vi "{TMPL} MAIN - App.vi"() -> ()   [LabVIEW 2023, in "TLB` InstStu GPlugin Template.lvlib" / "{TMPL} TLB`.lvclass"]
uses:
  {TMPL} TLB`.lvclass
  Application Components/Trigger API/System Trigger.ctl
  State Machine/State.ctl
  Core Components/Error Handler/TLB` Error Handler.lvclass
  Application Components/Configuration/{TMPL} Station Configuration.lvclass
  {TMPL} TLB`.lvclass/{TMPL} TLB`.ctl
  Application Components/InstStuGPluginSDK/Plugin Events.ctl
  Application Components/InstStuGPluginSDK/Plugin Events Enum.ctl
  <vilib>/Utility/error.llb/Error Cluster From Error Code.vi
  <vilib>/ErrorRing/Error Ring.xnode
  Application Components/Trigger API/{TMPL} Trigger API.lvlib
  TLB` InstStu GPlugin Template.lvlib
  Core Components/Actions/Actions.lvlib
  Core Components/Dependencies/TLB`_Dependencies.lvlib
  Application Components/UI/ScrollZoomGraphChart/ScrollZoomGraphChart.lvclass
  Application Components/InstStuGPluginSDK/Plugin Session.lvclass
  Application Components/InstStuGPluginSDK/InstrumentStudio Plugin SDK.lvlib
  <vilib>/Utility/LVLibp/NI_PackedLibraryUtility.lvlib
panel:
  in  "Session Id":u64
  out "top banner":u32(colorbox)=44412
  out "iq graph":waveform(sgl)[](graph) caption="Q Data"
  out "iq graph 2":waveform(sgl)[](graph) caption="Q Data"
  out "iq graph 3":waveform(sgl)[](graph) caption="Q Data"
  out "iq graph 4":waveform(sgl)[](graph) caption="Q Data"
  in  "RESOURCE NAME":refnum<visa-resource-name>
  in  "error":bool
  out "error background":u32(colorbox)=15461355
  in  "settings gear":bool
  in  "connect":bool
  in  "run":bool
  in  "single":bool
  out "title":string="INST STU GPLUGIN`"
  out "error out":errorcluster
  in  "digital offset":dbl caption="DIGITAL OFFSET" format="%1_3p"
  in  "digital gain":dbl=-10.0 caption="DIGITAL GAIN" format="%1_3p dB"
  in  "finite records?":bool=TRUE
  in  "iq rate":dbl=2160000000.0 caption="IQ  RATE" format="%1_6p samples/sec"
  in  "no of samples":u64=1000 caption="NO. SAMPLES"
  in  "no of records":u64=25 caption="NO. RECORDS"
  in  "finite samples?":bool=TRUE
  in  "acq sample rate":dbl=2160000000.0 caption="ACQ SAMPLE RATE" format="%1_6p samples/sec"
  out "State":string="<Shutdown> "
  out "Status":string
  # "Section  A"
  # "Section B"
  # "Category A"
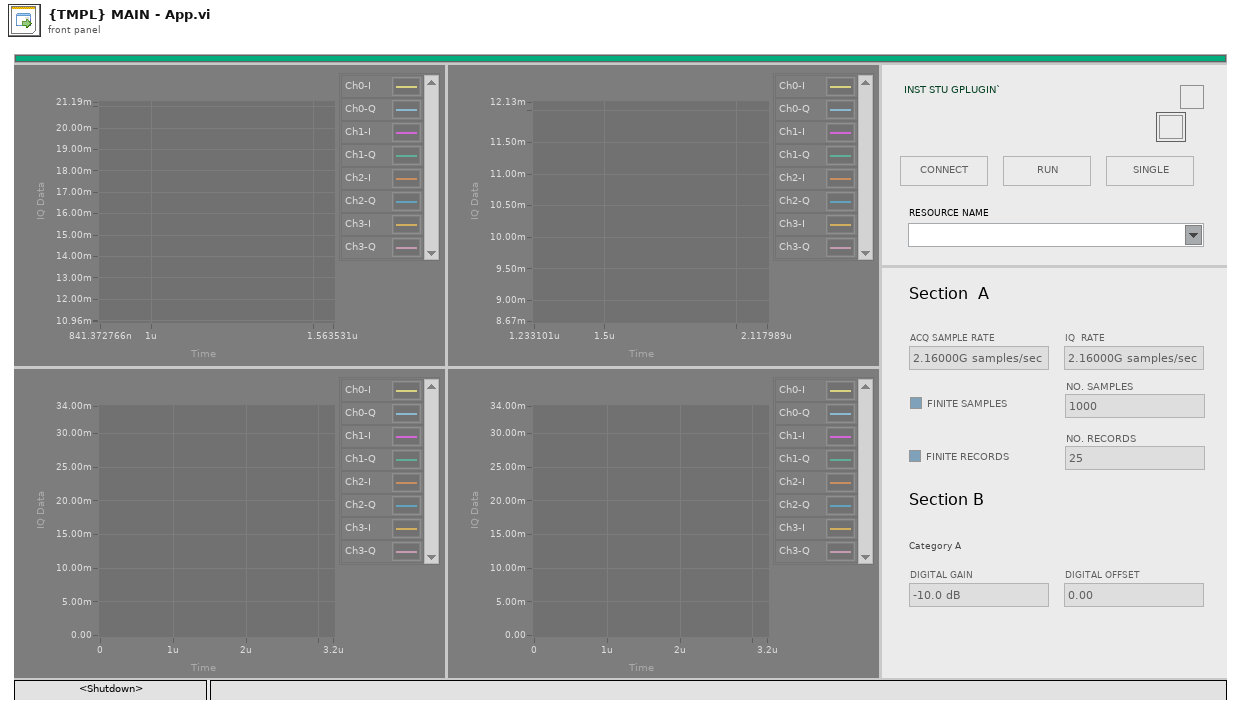
[diagram p1: front panel]
types:
  T1 = typedef "TLB` InstStu GPlugin Template.lvlib/{TMPL} TLB`.lvclass/State.ctl" = enum16{"<Startup>", "Idle", "Connected", "Monitoring", "<Shutdown>", "<Error>"}
  T2 = enum16{"Close Display", "Clear References", "Close Error Handler"}
  T3 = enum16{"Clear SR", "Set Display", "Set Shifter", "Initialize Events", "Init Q"}
  T4 = typedef "TLB` InstStu GPlugin Template.lvlib/{TMPL} Trigger API.lvlib/System Trigger.ctl" = enum16{"<None>", "Connect", "Start Acquisition", "Stop Acquisition", "Disconnect", "Load Configuration", "Save Configuration", "<Return to Safe State Actions>", "<Cache User Parameters>", "<Close Application>", "<Error>"}
  T5 = refnum<class "{TMPL} Station Configuration.lvclass">
  T6 = typedef "TLB` InstStu GPlugin Template.lvlib/InstrumentStudio Plugin SDK.lvlib/Plugin Events.ctl" = cluster{"Shutdown":refnum<user-event>, "Project Saved":refnum<user-event>, "Stop All Outputs":refnum<user-event>, "Generic Message":refnum<user-event>}
  T7 = typedef "TLB` InstStu GPlugin Template.lvlib/_UI CORE Event References.ctl" = cluster{"Exit Event":refnum<user-event>, "State Indicator":refnum<user-event>, "Status Indicator":refnum<user-event>}
  T8 = typedef "TLB` InstStu GPlugin Template.lvlib/_UI APP Event References.ctl" = cluster{"Exit Event":refnum<user-event>}
  T9 = typedef "TLB` InstStu GPlugin Template.lvlib/InstrumentStudio Plugin SDK.lvlib/Plugin Events Enum.ctl" = enum16{"Shutdown", "Project Saved", "Stop All Outputs", "Generic Message"}
  T10 = typedef "TLB` InstStu GPlugin Template.lvlib/InstrumentStudio Plugin SDK.lvlib/Panel Size.ctl" = enum32{"Large", "Small"}
  T11 = enum32{"Invalid", "Standard", "Closed", "Hidden", "Minimized", "Maximized"}
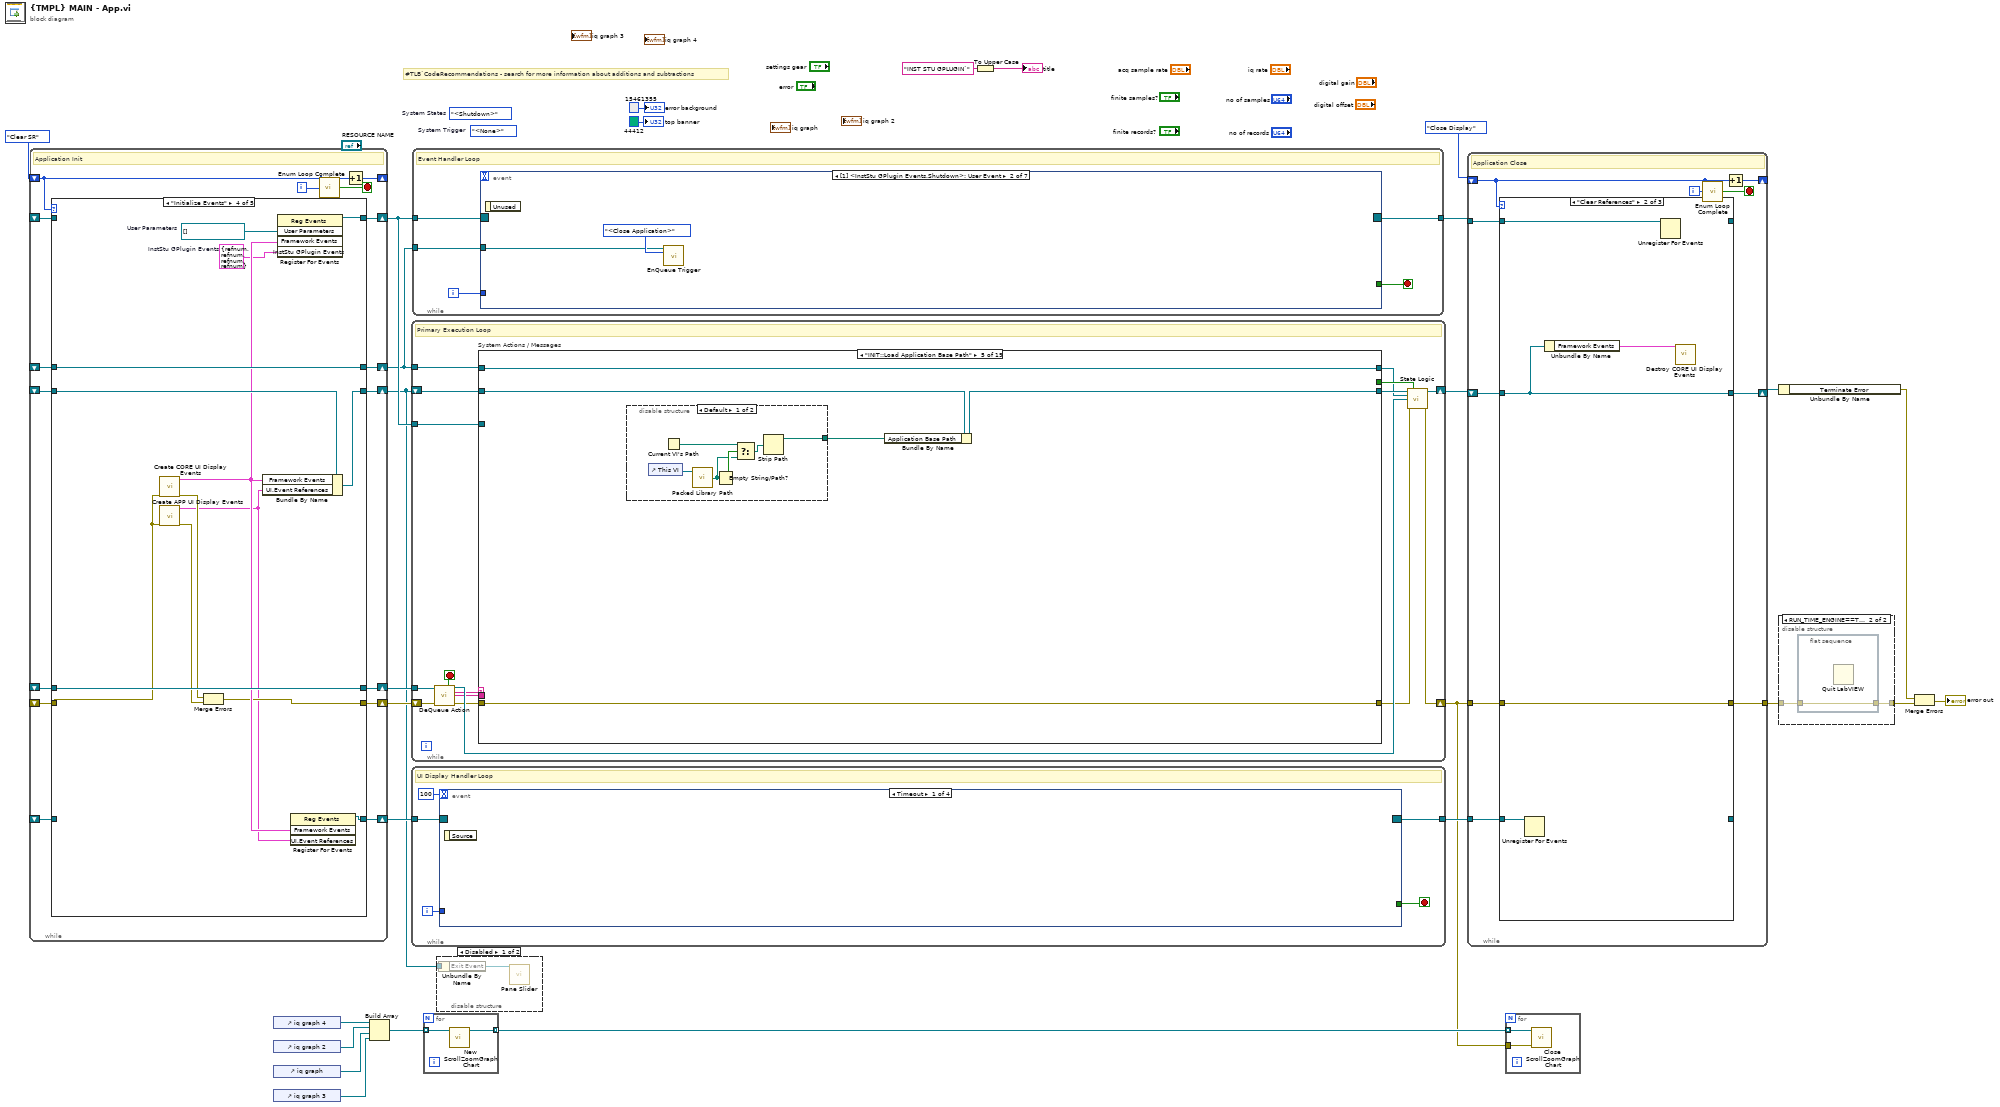
[diagram p0: block diagram]
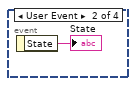
[diagram p3: hidden frame]
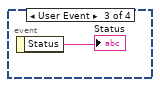
[diagram p4: hidden frame]
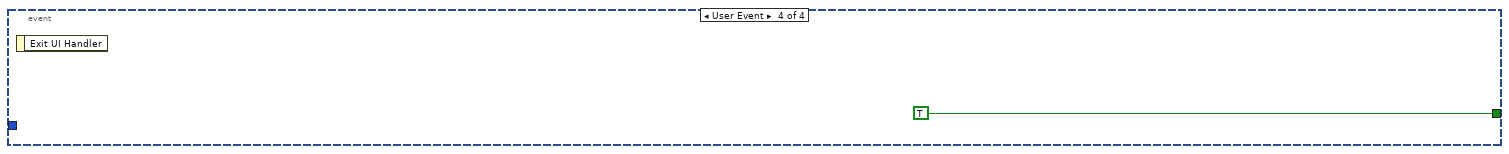
[diagram p5: hidden frame]
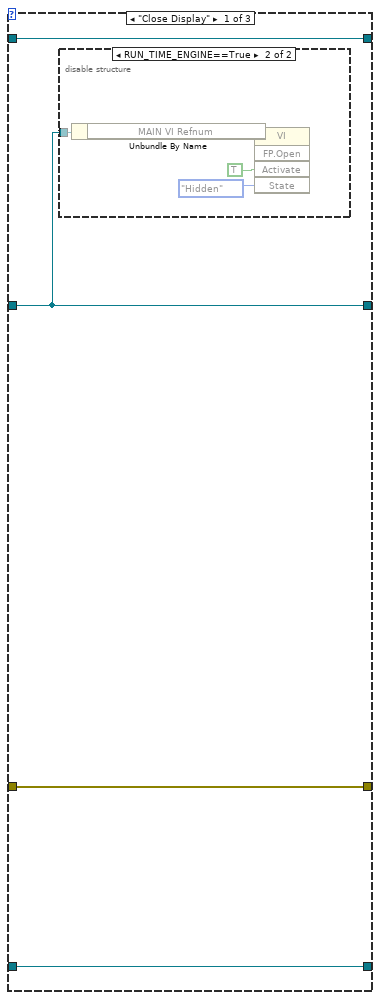
[diagram p7: hidden frame]
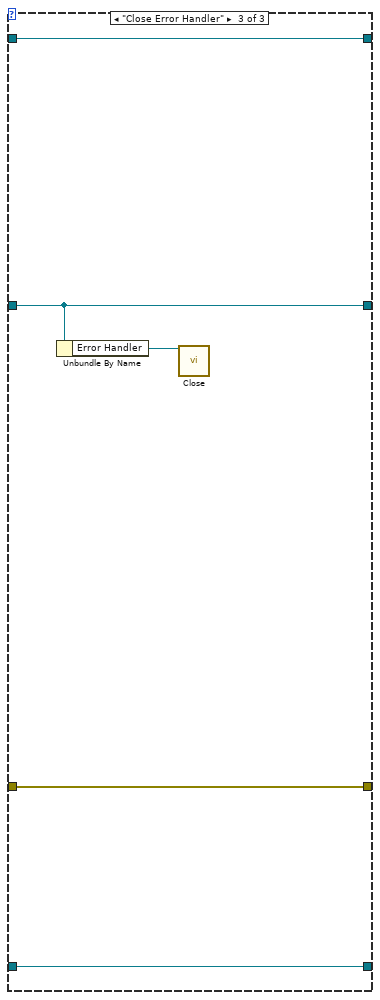
[diagram p9: hidden frame]
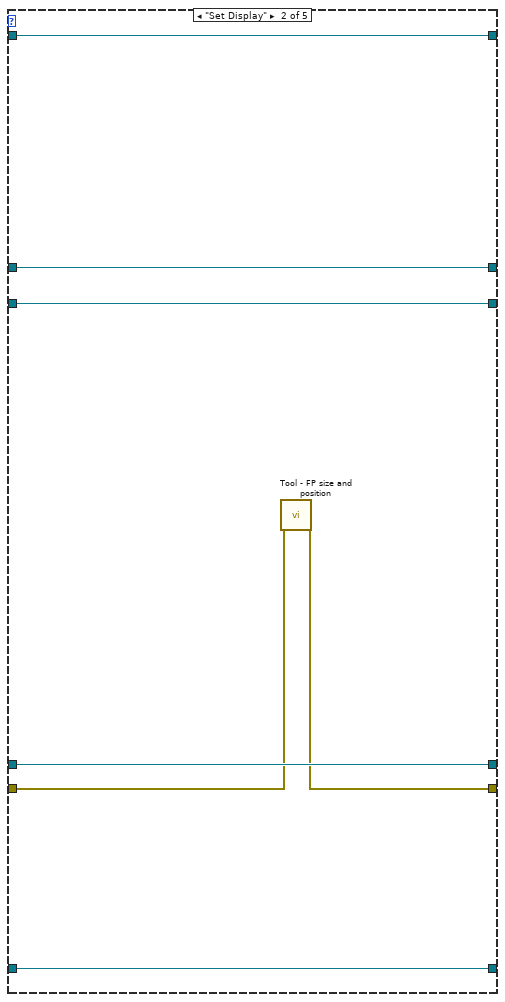
[diagram p11: hidden frame]
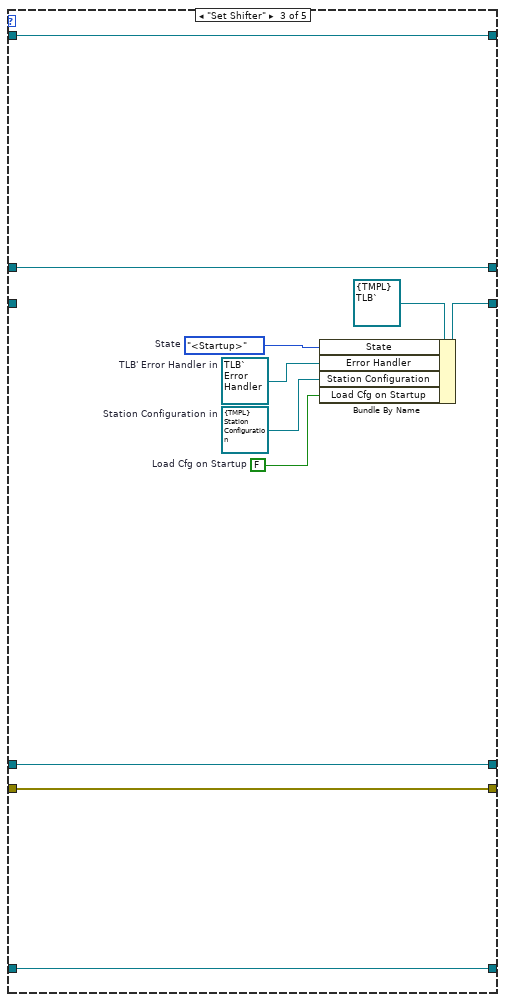
[diagram p12: hidden frame]
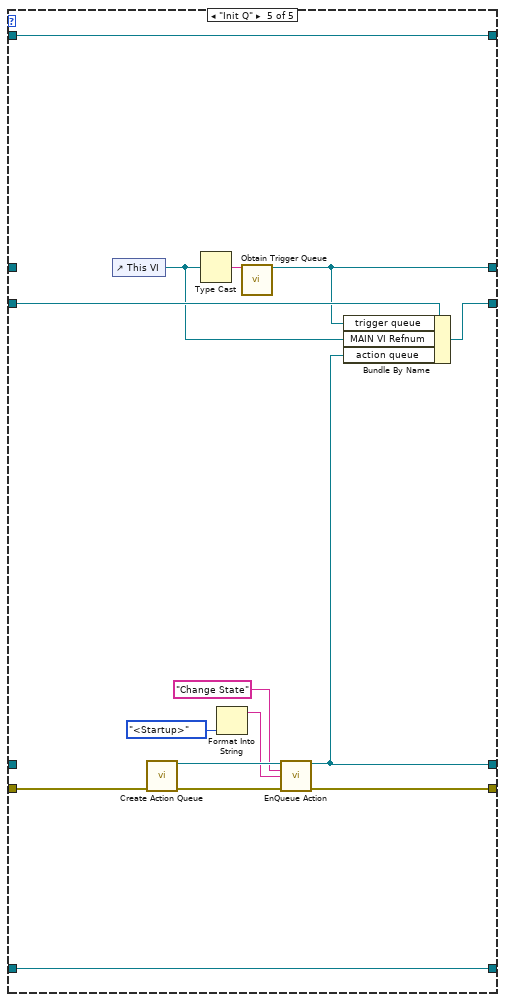
[diagram p13: hidden frame]
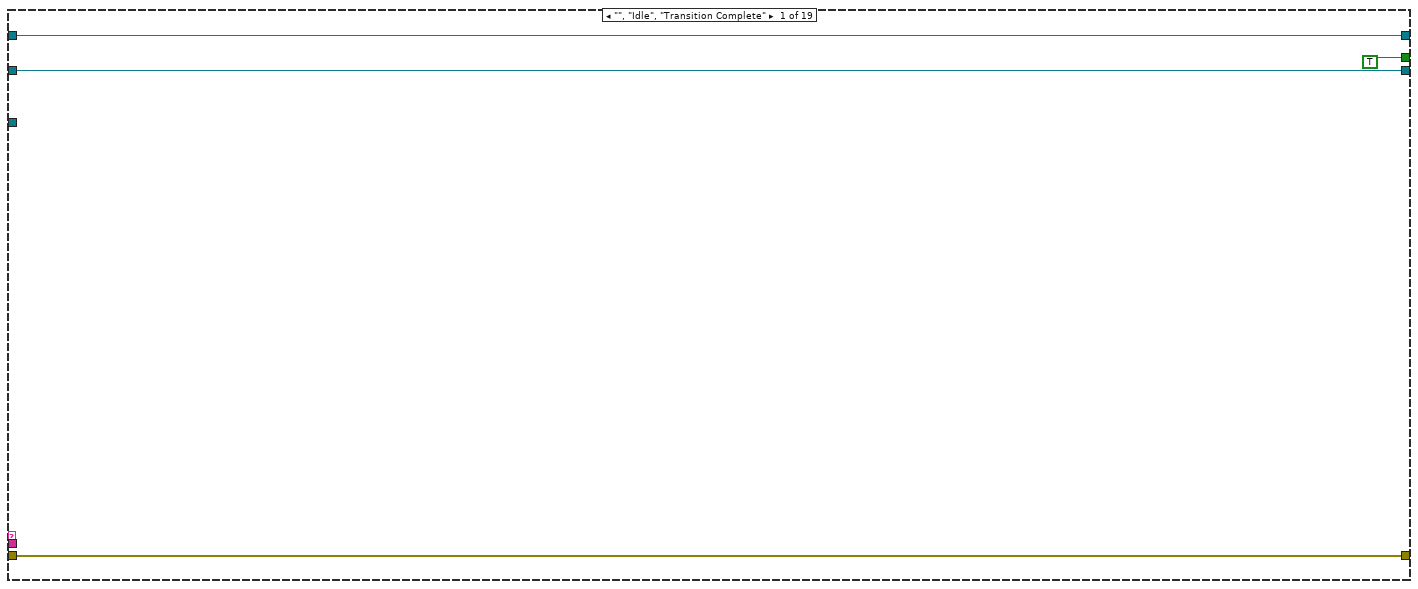
[diagram p14: hidden frame]
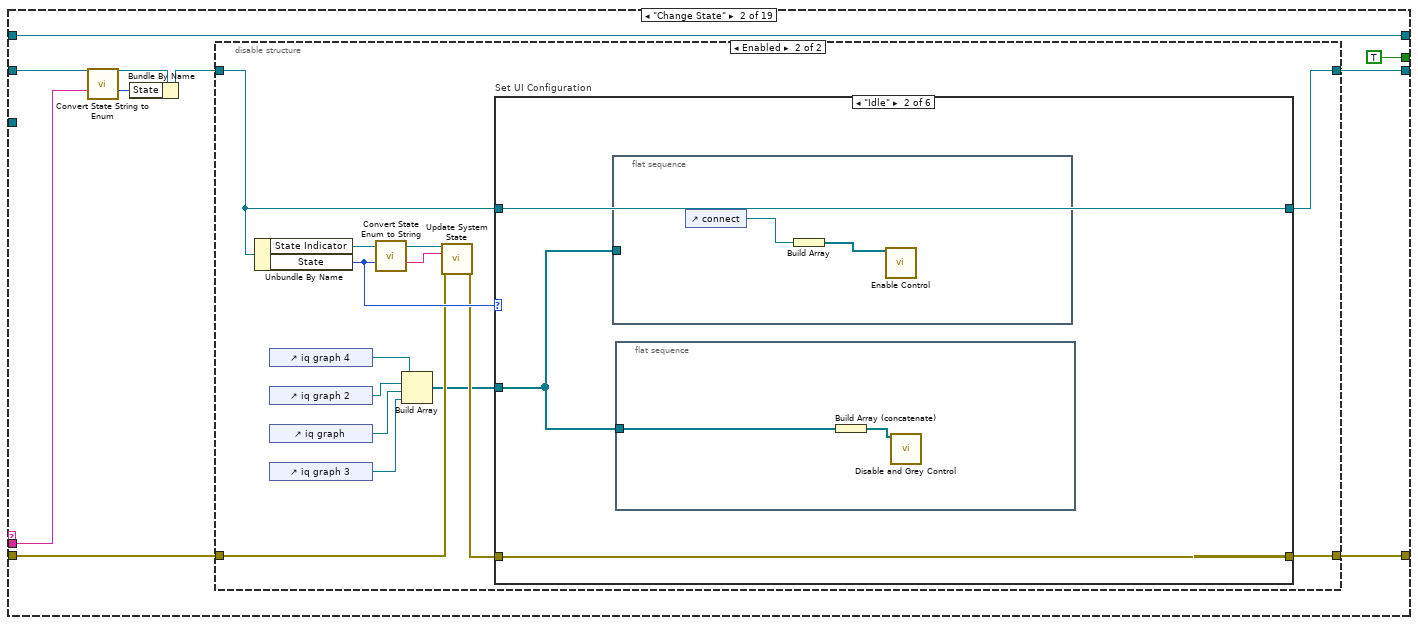
[diagram p15: hidden frame]
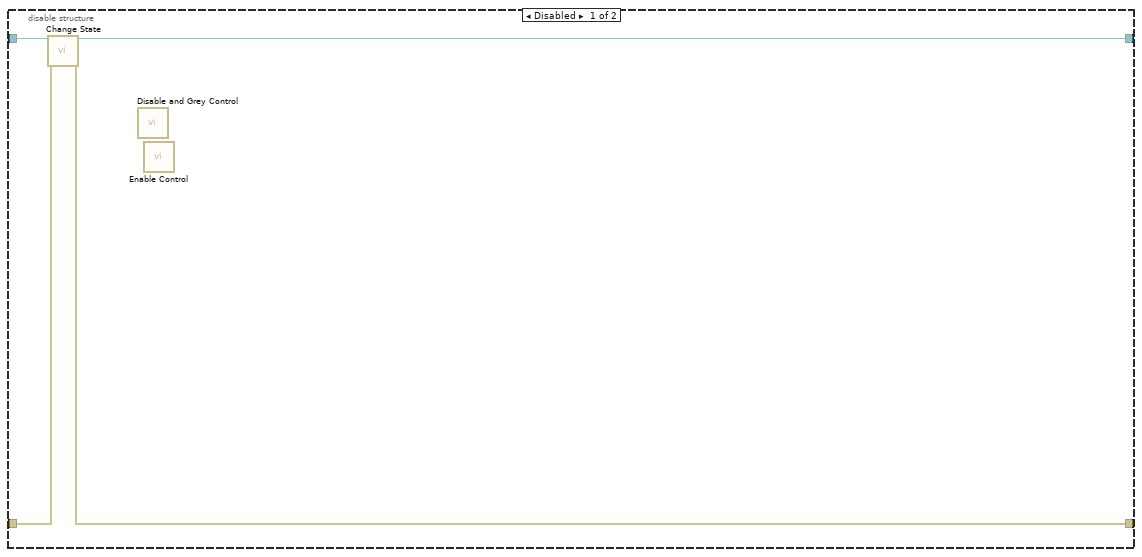
[diagram p16: hidden frame]
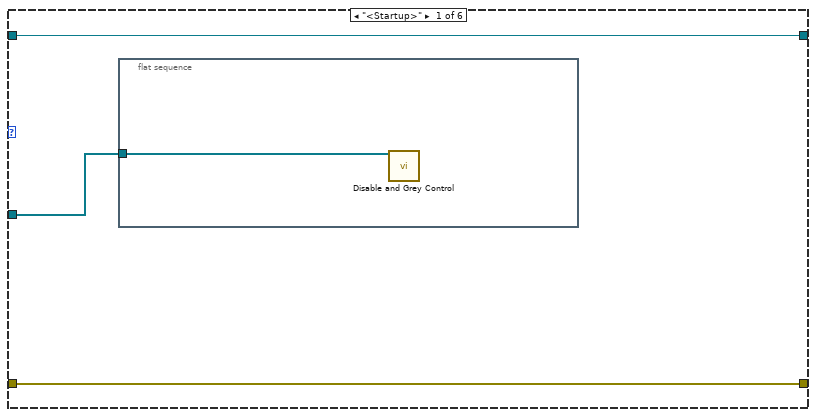
[diagram p17: hidden frame]
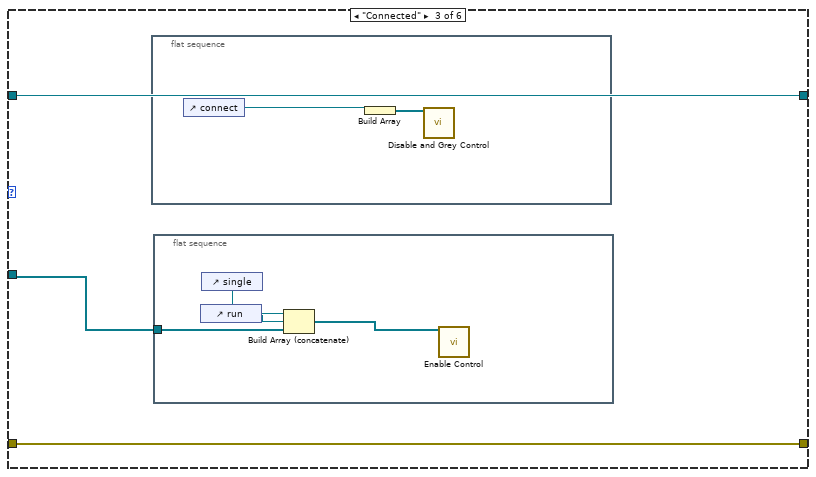
[diagram p18: hidden frame]
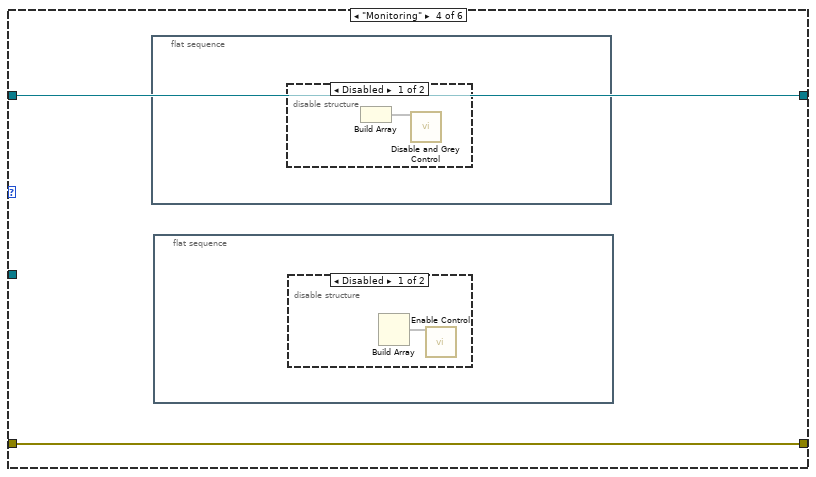
[diagram p19: hidden frame]
diagram:
  (unwired) State."<Shutdown>"  # System States
  (unwired) System_Trigger."<None>"  # System Trigger
  # "#TLB`CodeRecommendations - search for more information about additions and subtractions"
  n1 = while {
    shift-right: [w39] -> _
    shift-left: T3."Clear SR" -> [w28]
    shift-right: [w43] -> w27
    shift-left: _ -> [w38]
    shift-right: [w40] -> w22
    shift-left: _ -> [w37]
    shift-right: [w42] -> w21
    shift-left: _ -> [w36]
    shift-right: [w41] -> w12
    shift-left: _ -> [w35]
    shift-right: [w34] -> w18
    shift-left: _ -> [w33]
    shift-right: [w32] -> w20
    shift-left: _ -> [w31]
    i -> [w29]
    stop <- w30 stop-if-true
    # "Application Init"
    n2 = case shown="\"Initialize Events\"" w28 {
      tunnel: [_ w48 w61 w75 w76] -> w43
      tunnel: [_ w46 w60 w65 w82] -> w40
      tunnel: [_ w50 w56 w73 w88] -> w41
      tunnel: [_ w49 w59 w72 w90] -> w42
      tunnel: w38 -> [_ w48 w61 w75 _]
      tunnel: w37 -> [_ w47 w60 w64 w84]
      tunnel: w36 -> [_ w49 w59 _ w90]
      tunnel: w35 -> [_ w50 _ w74 w89]
      tunnel: [_ w45 w58 w71 w77] -> w34
      tunnel: w33 -> [_ w45 w58 w71 _]
      tunnel: [_ w44 w54 w69 w85] -> w32
      tunnel: w31 -> [_ w44 w54 _ w85]
      frame "Clear SR" {
      }
      frame "Set Display" {
        n3 = call "Tool - FP size and position.vi"("error in (no error)"=w47) -> ("error out"=w46:errorcluster)  [unwired: 17 in, 1 out]
      }
      frame "Set Shifter" {
        w51 = FALSE  # Load Cfg on Startup
        w52 = T5 refnum  # Station Configuration in
        w53 = refnum<class "TLB` Error Handler.lvclass"> refnum  # TLB' Error Handler in
        w57 = State."<Startup>"  # State
        n4 = Bundle By Name(cluster=refnum<class "{TMPL} TLB`.lvclass"> refnum ("TLB` Template.lvlib:TLB' Template.lvclass"), "State"=w57, "Error Handler"=w53, "Station Configuration"=w52, "Load Cfg on Startup"=w51) -> (w56:refnum<class "{TMPL} TLB`.lvclass">)
      }
      frame "Initialize Events" {
        w62 = T6 {"Shutdown"=refnum, "Project Saved"=refnum, "Stop All Outputs"=refnum, "Generic Message"=refnum}  # InstStu GPlugin Events
        w70 = refnum<vi>[] []  # User Parameters
        n5 = call "Create CORE UI Display Events.vi"("error in"=w64) -> ("Framework Events"=w68:T7, "error out"=w67:errorcluster)  [unwired: 13 in]
        n6 = call "Create APP UI Display Events.vi"("error in"=w64) -> ("UI.Event References"=w63:T8, "error out"=w66:errorcluster)  [unwired: 13 in]
        n7 = Merge Errors(w67, w66) -> (w65:errorcluster)
        n8 = Bundle By Name(cluster=w74, "Framework Events"=w68, "UI.Event References"=w63) -> (w73:refnum<class "{TMPL} TLB`.lvclass">)
        n9 = register-events(w70, w68, w62) -> (reference out=w72:refnum<event-registration>)  [unwired: 2 in, 1 out]
        n10 = register-events(w68, w63) -> (reference out=w69:refnum<event-registration>)  [unwired: 2 in, 1 out]
      }
      frame "Init Q" {
        n11 = control-ref of="This VI"() -> (w87:refnum<vi>)
        n12 = call "Create Action Queue.vi"("error in"=w84) -> ("action queue out"=w81:refnum<queue>, "error out"=w83:errorcluster)  [unwired: 13 in]
        n13 = Type Cast(x=w87) -> (*(type *) &x=w78:string)  [unwired: 1 in]
        n14 = Format Into String(State."<Startup>" ("State")) -> (resulting string=w79:string)  [unwired: 3 in, 1 out]
        n15 = call "Obtain Trigger Queue.vi"("trigger queue name"=w78) -> ("trigger queue out"=w77:refnum<queue>)  [unwired: 13 in, 1 out]
        n16 = call "EnQueue Action.vi"("action queue in"=w81, "action"="Change State" ("Message Name"), "data in"=w79, "error in"=w83) -> ("action queue out"=w76:refnum<queue>, "error out"=w82:errorcluster)  [unwired: 10 in]
        n17 = Bundle By Name(cluster=w89, "trigger queue"=w77, "MAIN VI Refnum"=w87, "action queue"=w76) -> (w88:refnum<class "{TMPL} TLB`.lvclass">)
      }
    }
    n18 = call "Enum Loop Complete.vi"("Current State Enum"=w28, "Itteration"=w29) -> ("Loop Complete?"=w30:bool)  [unwired: 12 in, 1 out]
    n19 = Increment(x=w28) -> (x+1=w39:T3)
  }
  n20 = control-ref of="iq graph 4"() -> (w7:refnum<vi>)
  n21 = control-ref of="iq graph 2"() -> (w5:refnum<vi>)
  n22 = control-ref of="iq graph"() -> (w4:refnum<vi>)
  n23 = control-ref of="iq graph 3"() -> (w3:refnum<vi>)
  n24 = Build Array(w7, w5, w4, w3) -> (w6:refnum<vi>[])
  n25 = while {
    shift-right: [w101] -> w1
    shift-left: w22 -> [w96]
    shift-right: [w103] -> w23
    shift-left: w12 -> [w105]
    tunnel: w27 -> [w97]
    tunnel: w21 -> [w104]
    tunnel: w18 -> [w100]
    stop <- w95 stop-if-true
    # "Primary Execution Loop"
    n26 = call "DeQueue Action.vi"("action queue in"=w97, "error in"=w96) -> ("exit?"=w95:bool, "action queue out"=w106:refnum<queue>, "action"=w93:string, "action value"=w91:string, "error out"=w94:errorcluster)  [unwired: 8 in, 1 out]
    n27 = case "System Actions / Messages" shown="\"INIT::Load Application Base Path\"" w93 {
      selector: w93 -> [_ _ _ _ _ _ _ _ _ _ _ _ _ _ _ _ _ _ w290]
      tunnel: [w110 w117 w178 w185 w186 w199 w208 w226 w238 w241 w248 w254 w257 w260 w267 w272 w273 w285 w289] -> w98
      tunnel: w94 -> [w110 w116 w178 w185 w186 w202 w208 w225 w238 w241 w246 w254 w257 w260 w266 w272 w274 w286 _]
      tunnel: w105 -> [w107 w115 w176 w184 w189 w200 w211 w232 w237 w239 w242 w253 w256 w259 w269 w271 w277 w288 w292]
      tunnel: [w107 w111 w179 w184 w188 w205 w214 w224 w237 w239 w243 w253 w256 w259 w269 w271 w276 w287 w292] -> w102
      tunnel: w104 -> [_ _ _ _ _ _ w212 w233 _ _ _ _ _ _ _ _ _ _ _]
      tunnel: [w108 w118 w177 w183 w190 w206 w213 w234 w236 w240 w251 w252 w255 w258 w264 w270 w280 w281 w291] -> w92
      tunnel: w100 -> [w108 w118 w177 w183 w190 w206 w213 w234 w236 w240 w251 w252 w255 w258 w264 w270 w280 w281 w291]
      tunnel: [TRUE TRUE _ _ _ _ _ _ _ _ _ _ _ _ _ _ _ _ _] -> w99
      tunnel: w91 -> [_ w114 _ _ _ _ _ _ _ _ _ _ _ _ _ _ _ _ _]
      frame "", "Idle", "Transition Complete" {
      }
      frame "Change State" {
        n28 = call "Convert State String to Enum.vi"("state in"=w114) -> ("state out"=w113:T1)  [unwired: 13 in, 1 out]
        n29 = Bundle By Name(cluster=w115, "State"=w113) -> (w112:refnum<class "{TMPL} TLB`.lvclass">)
        n30 = disable-structure shown="Enabled" {
          disable-tunnel: [w123 w129] -> w117
          disable-tunnel: w116 -> [w122 w130]
          disable-tunnel: w112 -> [w121 w132]
          disable-tunnel: [w120 w131] -> w111
          frame Disabled {
            n31 = call "Change State.vi"("TLB' data in"=w121, "error in"=w122) -> ("TLB' data out"=w120:refnum<class "{TMPL} TLB`.lvclass">, "error out"=w123:errorcluster)  [unwired: 12 in]
            n32 = call "Disable and Grey Control.vi"() -> ()  [unwired: 15 in, 1 out]
            n33 = call "Enable Control.vi"() -> ()  [unwired: 15 in, 1 out]
          }
          frame Enabled {
            n34 = Unbundle By Name(w132) -> ("State Indicator"=w133:refnum<user-event>, "State"=w136:T1)
            n35 = control-ref of="iq graph 4"() -> (w128:refnum<vi>)
            n36 = control-ref of="iq graph 2"() -> (w127:refnum<vi>)
            n37 = control-ref of="iq graph"() -> (w126:refnum<vi>)
            n38 = control-ref of="iq graph 3"() -> (w125:refnum<vi>)
            n39 = call "Convert State Enum to String.vi"("state in"=w136) -> ("state out"=w134:string)  [unwired: 13 in, 1 out]
            n40 = Build Array(w128, w127, w126, w125) -> (w124:refnum<vi>[])
            n41 = call "Update System State.vi"("State Indicator"=w133, "system state message"=w134, "error in"=w130) -> ("error out"=w135:errorcluster)  [unwired: 12 in]
            n42 = case "Set UI Configuration" shown="\"Idle\"" w136 {
              tunnel: [w138 w143 w150 w158 w169 w174] -> w129
              tunnel: w135 -> [w138 w143 w150 w158 w169 w174]
              tunnel: [w139 w142 w149 w157 w168 w175] -> w131
              tunnel: w132 -> [w139 w142 w149 w157 w168 w175]
              tunnel: w124 -> [w137 w141 w148 _ w167 _]
              frame "<Startup>" {
                n43 = flat-sequence {
                  tunnel: w137 -> [w140]
                  frame #0 {
                    n44 = call "Disable and Grey Control.vi"("Control Ref"=w140) -> ()  [unwired: 14 in, 1 out]
                  }
                }
              }
              frame "Idle" {
                n45 = flat-sequence {
                  tunnel: w141 -> [_]
                  frame #0 {
                    n46 = control-ref of="connect"() -> (w146:refnum<vi>)
                    n47 = Build Array(w146) -> (w147:refnum<vi>[])
                    n48 = call "Enable Control.vi"("Control Ref"=w147) -> ()  [unwired: 14 in, 1 out]
                  }
                }
                n49 = flat-sequence {
                  tunnel: w141 -> [w145]
                  frame #0 {
                    n50 = Build Array (concatenate)(w145) -> (w144:refnum<vi>[])
                    n51 = call "Disable and Grey Control.vi"("Control Ref"=w144) -> ()  [unwired: 14 in, 1 out]
                  }
                }
              }
              frame "Connected" {
                n52 = flat-sequence {
                  frame #0 {
                    n53 = control-ref of="connect"() -> (w156:refnum<vi>)
                    n54 = Build Array(w156) -> (w155:refnum<vi>[])
                    n55 = call "Disable and Grey Control.vi"("Control Ref"=w155) -> ()  [unwired: 14 in, 1 out]
                  }
                }
                n56 = flat-sequence {
                  tunnel: w148 -> [w154]
                  frame #0 {
                    n57 = control-ref of="run"() -> (w151:refnum<vi>)
                    n58 = control-ref of="single"() -> (w152:refnum<vi>)
                    n59 = Build Array (concatenate)(w152, w151, w154) -> (w153:refnum<vi>[])
                    n60 = call "Enable Control.vi"("Control Ref"=w153) -> ()  [unwired: 14 in, 1 out]
                  }
                }
              }
              frame "Monitoring" {
                n61 = flat-sequence {
                  frame #0 {
                    n62 = disable-structure shown="Disabled" {
                      frame Disabled {
                        n63 = Build Array() -> (w165:void[], w166:dbl, w164:dbl)
                        n64 = call "Disable and Grey Control.vi"("Control Ref"=w165) -> ()  [unwired: 14 in, 1 out]
                      }
                      frame Enabled {
                      }
                    }
                  }
                }
                n65 = flat-sequence {
                  frame #0 {
                    n66 = disable-structure shown="Disabled" {
                      frame Disabled {
                        n67 = Build Array() -> (w160:void[], w163:dbl, w159:dbl, w162:dbl, w161:dbl)
                        n68 = call "Enable Control.vi"("Control Ref"=w160) -> ()  [unwired: 14 in, 1 out]
                      }
                      frame Enabled {
                      }
                    }
                  }
                }
              }
              frame "<Shutdown>" {
                n69 = flat-sequence {
                  tunnel: w167 -> [w173]
                  frame #0 {
                    n70 = control-ref of="run"() -> (w170:refnum<vi>)
                    n71 = control-ref of="single"() -> (w171:refnum<vi>)
                    n72 = Build Array (concatenate)(w171, w170, w173) -> (w172:refnum<vi>[])
                    n73 = call "Disable and Grey Control.vi"("Control Ref"=w172) -> ()  [unwired: 14 in, 1 out]
                  }
                }
              }
              frame "<Error>" {
              }
            }
          }
        }
      }
      frame "Cache User Parameters" {
        n74 = disable-structure "<Add Your User Parameter Terminals Here>" shown="Disabled" {
          disable-tunnel: [w181 w182] -> w179
          disable-tunnel: w176 -> [w180 w182]
          frame Disabled {
            n75 = Bundle By Name(cluster=w180) -> (w181:refnum<class "{TMPL} TLB`.lvclass">)  [unwired: 2 in]
          }
          frame Enabled {
          }
        }
      }
      frame "/*********INITialize********/" {
      }
      frame "INIT::Load Application Base Path" {
        n76 = disable-structure shown="Default" {
          disable-tunnel: [w195 w197] -> w187
          frame condition #0 (active) {
            n77 = control-ref of="This VI"() -> (w194:refnum<vi>)
            n78 = Current VI's Path() -> (path=w196:path)
            n79 = call <vilib>:"Packed Library Path.vi"("vi reference"=w194) -> ("packed library path"=w191:path)  [unwired: 2 in, 2 out]
            n80 = Empty String/Path?(string/path=w191) -> (empty?=w192:bool)
            n81 = Select(t=w196, s=w192, f=w191) -> (s? t:f=w193:path)
            n82 = Strip Path(path=w193) -> (stripped path=w195:path)  [unwired: 1 out]
          }
          frame condition #1 {
            n83 = call <vilib>:"Application Directory.vi"() -> ("Application Directory"=w197:path)
          }
        }
        n84 = Bundle By Name(cluster=w189, "Application Base Path"=w187) -> (w188:refnum<class "{TMPL} TLB`.lvclass">)
      }
      frame "INIT::Initialize Error Handler" {
        n85 = Unbundle By Name(w200) -> ("Application Base Path"=w207:path)
        n86 = Unbundle By Name(w200) -> ("Error Handler"=w201:refnum<class "TLB` Error Handler.lvclass">)
        n87 = Build Path(base path=w207, name or relative path="System Level Errors\\System Errors.txt") -> (appended path=w203:path)
        n88 = call-dynamic "Open.vi"("error handler in"=w201, "error log path in"=w203, "error in"=w202) -> ("error handler out"=w204:refnum<class "TLB` Error Handler.lvclass">, "error out"=w199:errorcluster)  [unwired: 11 in]
        n89 = Bundle By Name(cluster=w200, "Error Handler"=w204) -> (w205:refnum<class "{TMPL} TLB`.lvclass">)
      }
      frame "INIT::Register User Parameters" {
        n90 = disable-structure shown="Enabled" {
          disable-tunnel: [w215 refnum<vi>[] [] ("User Parameter Controls")] -> w210
          frame Disabled {
            n91 = stacked-sequence "Stacked Sequence Structure :: Allows for a lot of controls" {
              tunnel: [w218] -> w215
              frame #0 {
                n92 = Build Array() -> (w218:void[], w217:dbl, w216:dbl)
              }
            }
          }
          frame Enabled {
          }
        }
        n93 = Build Array (concatenate)(w210) -> (w209:refnum<vi>[])
        n94 = register-events(reference=w212, w209) -> ()  [unwired: 3 in, 2 out]
        n95 = Bundle By Name(cluster=w211, "User Parameter Controls"=w209) -> (w214:refnum<class "{TMPL} TLB`.lvclass">)
      }
      frame "INIT::Register Instrument Studio" {
        w227 = T9[] [enum."Shutdown", enum."Project Saved", enum."Stop All Outputs", enum."Generic Message"] items=["Shutdown", "Project Saved", "Stop All Outputs", "Generic Message"] ("Events To Register")
        n96 = call "Create Session.vi"("error in (no error)"=w225, "Session Id"="Session Id") -> ("error out"=w228:errorcluster, "Run Time Configuration"=w220:string, "Edit Time Configuration"=w221:string, "Session out"=w230:refnum<class "Plugin Session.lvclass">, "Panel Size"=w222:T10)  [unwired: 5 in]
        n97 = call "Register For Events.vi"("error in (no error)"=w228, "Events To Register"=w227, "Session in"=w230) -> ("error out"=w235:errorcluster, "Plugin Events"=w229:T6, "Session out"=w223:refnum<class "Plugin Session.lvclass">)  [unwired: 5 in, 1 out]
        n98 = register-events(reference=w233, error in=w235, w229) -> (error out=w226:errorcluster)  [unwired: 2 in, 1 out]
        n99 = Bundle By Name(cluster=w232, "InstStu GPlugin"=w223, "Panel Size"=w222, "Edit Time Configuration"=w221, "Run Time Configuration"=w220) -> (w224:refnum<class "{TMPL} TLB`.lvclass">)
      }
      frame "INIT::FP Values" {
        # "#TLB`CodeRecommendations - initialize FP values here"
      }
      frame "INIT::Initialize System Parameters" {
      }
      frame "CFG::Load Station Configuration" {
        n100 = Unbundle By Name(w242) -> ("Station Configuration"=w245:T5)
        n101 = Unbundle By Name(w242) -> ("Application Base Path"=w250:path)
        n102 = Build Path(base path=w250, name or relative path="System Configuration\\Station Configuration.ini") -> (appended path=w247:path)
        n103 = call-dynamic "Load Configuration.vi"("INI Station Configuration in"=w245, "INI file path in"=w247, "error in"=w246) -> ("INI Station Configuration out"=w244:T5, "error out"=w248:errorcluster)  [unwired: 11 in]
        n104 = Bundle By Name(cluster=w242, "Station Configuration"=w244) -> (w243:refnum<class "{TMPL} TLB`.lvclass">)
      }
      frame "/*********PRImary EXEcution********/" {
      }
      frame "APP::Update Display" {
      }
      frame "/*********SHUTDOWN********/" {
      }
      frame "Exit" {
        w265 = refnum<class> refnum  # event data
        # "Don't wire 'Error In'\nMust Execute Regardless"
        n105 = Unbundle By Name(w269) -> ("Exit Event"=w263:refnum<user-event>, "InstStu GPlugin"=w262:refnum<class "Plugin Session.lvclass">)
        n106 = Generate User Event(user event=w263, event data cluster=w265) -> (error out=w268:errorcluster)  [unwired: 2 in, 1 out]
        n107 = call "Close Session.vi"("Session in"=w262) -> ("error out"=w261:errorcluster)  [unwired: 10 in]
        n108 = Merge Errors(w266, w268, w261) -> (w267:errorcluster)
      }
      frame "/*********ERRor Handler********/" {
      }
      frame "ERR::Log" {
        n109 = Unbundle By Name(w277) -> ("Error Handler"=w279:refnum<class "TLB` Error Handler.lvclass">)
        n110 = call-dynamic "Log.vi"("error handler in"=w279) -> ("error handler out"=w278:refnum<class "TLB` Error Handler.lvclass">, "error out"=w275:errorcluster)  [unwired: 13 in]
        n111 = Bundle By Name(cluster=w277, "Error Handler"=w278) -> (w276:refnum<class "{TMPL} TLB`.lvclass">)
        n112 = Merge Errors(w274, w275) -> (w273:errorcluster)
      }
      frame "ERR::Dialog" {
        n113 = Unbundle By Name(w288) -> ("Error Handler"=w284:refnum<class "TLB` Error Handler.lvclass">)
        n114 = call-dynamic "Dialog.vi"("error handler in"=w284, "trigger queue in"=w281) -> ("error handler out"=w283:refnum<class "TLB` Error Handler.lvclass">, "error out"=w282:errorcluster)  [unwired: 12 in]
        n115 = Merge Errors(w286, w282) -> (w285:errorcluster)
        n116 = Bundle By Name(cluster=w288, "Error Handler"=w283) -> (w287:refnum<class "{TMPL} TLB`.lvclass">)
      }
      frame Default {
        n117 = xnode "Error Ring"("parameter 0"=w290) -> ("error out"=w289:errorcluster)
      }
    }
    n118 = call "State Logic.vi"("TLB' data in"=w102, "process state logic enable"=w99, "trigger queue in"=w92, "action queue in"=w106, "error in"=w98) -> ("TLB' data out"=w103:refnum<class "{TMPL} TLB`.lvclass">, "error out"=w101:errorcluster)  [unwired: 9 in]
  }
  n119 = while {
    tunnel: w20 -> [w304]
    tunnel: [w300] -> w19
    i -> [w303]
    stop <- w302 stop-if-true
    # "UI Display Handler Loop"
    n120 = event shown="[0] Timeout" {
      selector: w304 -> [_ _ _ _]
      dyn-events: [_ _ _ _] -> w300
      timeout: 100 -> [_ _ _ _]
      tunnel: w303 -> [_ _ _ _]
      tunnel: [_ _ _ TRUE] -> w302
      event Timeout {
        n121 = event-data() -> ()  [unwired: 2 out]
      }
      event User Event {
        n122 = event-data() -> ("State"=→"State":string)  [unwired: 1 out]
      }
      event User Event {
        n123 = event-data() -> ("Status"=→"Status":string)  [unwired: 1 out]
      }
      event User Event {
        n124 = event-data() -> ()  [unwired: 2 out]
      }
    }
  }
  n125 = while {
    tunnel: w21 -> [w311]
    tunnel: [w310] -> w24
    tunnel: w18 -> [w308]
    i -> [w309]
    stop <- w312 stop-if-true
    # "Event Handler Loop"
    n126 = event shown="[1] <InstStu GPlugin Events.Shutdown>: User Event" {
      selector: w311 -> [_ _ _ _ _ _ _]
      dyn-events: [_ _ _ _ _ _ _] -> w310
      timeout: _ -> [_ _ _ _ _ _ _]
      tunnel: [_ _ _ TRUE ("NewVal") _ _ _] -> w312
      tunnel: w309 -> [_ _ _ _ _ _ _]
      tunnel: w308 -> [w313 w316 _ w339 w343 w346 w352]
      event Panel Close? {
        w315 = TRUE  # Discard?
        n127 = event-data() -> ()  [unwired: 2 out]
        n128 = call "EnQueue Trigger.vi"("trigger queue in"=w313, "system trigger"=System_Trigger."<Close Application>" ("System Trigger")) -> ()  [unwired: 12 in, 2 out]
        n129 = event-data("Discard?"=w315) -> ()  [unwired: 1 in, 1 out]
      }
      event User Event {
        n130 = event-data() -> ()  [unwired: 2 out]
        n131 = call "EnQueue Trigger.vi"("trigger queue in"=w316, "system trigger"=System_Trigger."<Close Application>" ("System Trigger")) -> ()  [unwired: 12 in, 2 out]
      }
      event "top banner": Mouse Up {
        n132 = event-data() -> ("Button"=w318:u16, "Mods.Double Click"=w319:bool)  [unwired: 1 out]
        n133 = Equal?(x=u16 2, y=w318) -> (x = y?=w321:bool)
        n134 = Compound Arithmetic op=AND(w321, w319) -> (w320:bool)
        n135 = case "Toggle Menu Visibility :: double RIGHT click on logo" shown="True" w320 {
          frame False {
          }
          frame True {
            n136 = First Call?() -> (First Call?: T/F=w327:bool)
            n137 = feedback #1() -> (w325:bool)  [unwired: 1 in]
            n138 = feedback #2() -> (w326:bool)  [unwired: 1 in]
            n139 = case shown="False" w327 {
              tunnel: [w331 w337] -> w329
              tunnel: [w330 w336] -> w328
              tunnel: w326 -> [w333 _]
              tunnel: w325 -> [w332 _]
              tunnel: [w333 TRUE] -> w324
              tunnel: [w332 TRUE] -> w323
              frame False {
                n140 = Not(x=w333) -> (.not. x?=w331:bool)
                n141 = Not(x=w332) -> (.not. x?=w330:bool)
              }
              frame True {
                n142 = property class="VI"() -> ("TB.Visible"=w337:bool, "Front Panel.ShowMenuBar"=w336:bool)  [unwired: 2 in, 2 out]
              }
            }
            n143 = feedback-in #1(w328) -> ()
            n144 = feedback-in #2(w329) -> ()
            n145 = property class="VI"("TB.Visible"=w324, "Front Panel.ShowMenuBar"=w323) -> ()  [unwired: 2 in, 2 out]
          }
        }
      }
      event User Event {
        n146 = event-data() -> ()  [unwired: 2 out]
        n147 = call "EnQueue Trigger.vi"("trigger queue in"=w339, "system trigger"=System_Trigger."<Close Application>" ("System Trigger")) -> ()  [unwired: 12 in, 2 out]
      }
      event Value Change {
        n148 = event-data() -> ()  [unwired: 2 out]
        n149 = call "EnQueue Trigger.vi"("trigger queue in"=w343, "system trigger"=System_Trigger."<Cache User Parameters>" ("System Trigger")) -> ("trigger queue out"=w342:refnum<queue>)  [unwired: 12 in, 1 out]
        n150 = event "use this event case to register a SPEICIFIC 'User Parameter' for a SPECIFIC action" shown="[0] Timeout" {
          selector: _ -> [_]
          dyn-events: _ -> [_]
          timeout: 0 -> [_]
          tunnel: w342 -> [_]
          event Timeout {
            n151 = event-data() -> ()  [unwired: 1 in, 1 out]
          }
        }
      }
      event "connect": Value Change {
        n152 = event-data() -> ()  [unwired: 2 out]
        n153 = call "EnQueue Trigger.vi"("trigger queue in"=w346, "system trigger"=System_Trigger."Connect" ("System Trigger")) -> ()  [unwired: 12 in, 2 out]
      }
      event "single": Value Change {
        n154 = event-data() -> ()  [unwired: 2 out]
        n155 = Select(t="runonce", s="single", f="") -> (s? t:f=w347:string)
        n156 = call "EnQueue Trigger.vi"("trigger queue in"=w352, "system trigger"=System_Trigger."Start Acquisition" ("System Trigger"), "trigger data"=w347) -> ()  [unwired: 11 in, 2 out]
      }
    }
  }
  n157 = for {
    tunnel: w6 -> [w354] mode=indexing
    tunnel: [w353] -> w2 mode=indexing
    n158 = call "New ScrollZoomGraphChart.vi"("Reference"=w354) -> ("ScrollZoomGraphChart out"=w353:refnum<class "ScrollZoomGraphChart.lvclass">)  [unwired: 9 in, 1 out]
  }
  n159 = disable-structure shown="Disabled" {
    disable-tunnel: w12 -> [w357 _]
    frame Disabled {
      n160 = Unbundle By Name(w357) -> ("Exit Event"=w356:refnum<user-event>)
      n161 = call "Pane Slider.vi"("User Event in"=w356) -> ("Invoke Button"=w355:refnum<vi>)  [unwired: 14 in]
    }
    frame Enabled {
    }
  }
  n162 = To Upper Case(1:"INST STU GPLUGIN`" ("title")) -> (0:→"title":string)
  n163 = while {
    shift-right: [w367] -> _
    shift-left: T2."Close Display" -> [w360]
    tunnel: w24 -> [w365]
    tunnel: w1 -> [w366]
    tunnel: [w363] -> w26
    shift-right: [w362] -> w16
    shift-left: w23 -> [w364]
    tunnel: w19 -> [w361]
    i -> [w358]
    stop <- w359 stop-if-true
    # "Application Close"
    n164 = case shown="\"Clear References\"" w360 {
      tunnel: [w370 w380 w385] -> w363
      tunnel: [w369 w379 w382] -> w362
      tunnel: [w371 _ w384] -> _
      tunnel: w366 -> [w370 w380 w385]
      tunnel: w365 -> [w371 w378 w384]
      tunnel: w364 -> [w369 w379 w382]
      tunnel: w361 -> [w368 w376 w383]
      tunnel: [w368 _ w383] -> _
      frame "Close Display" {
        n165 = disable-structure shown="RUN_TIME_ENGINE==True" {
          disable-tunnel: w369 -> [_ w373]
          frame condition #0 (active) {
          }
          frame condition #1 {
            n166 = Unbundle By Name(w373) -> ("MAIN VI Refnum"=w372:refnum<vi>)
            n167 = invoke class="VI" method="FP.Open"(reference=w372, "Activate"=TRUE ("Activate?"), "State"=T11."Hidden") -> ()  [unwired: 2 in, 5 out]
          }
        }
      }
      frame "Clear References" {
        n168 = Unregister For Events(event registration refnum=w376) -> ()  [unwired: 1 in, 1 out]
        n169 = Unbundle By Name(w379) -> ("Framework Events"=w377:T7)
        n170 = Unregister For Events(event registration refnum=w378) -> ()  [unwired: 1 in, 1 out]
        n171 = call "Destroy CORE UI Display Events.vi"("UI display events in"=w377) -> ()  [unwired: 14 in, 1 out]
      }
      frame "Close Error Handler" {
        n172 = Unbundle By Name(w382) -> ("Error Handler"=w381:refnum<class "TLB` Error Handler.lvclass">)
        n173 = call-dynamic "Close.vi"("error handler in"=w381) -> ()  [unwired: 14 in, 1 out]
      }
    }
    n174 = call "Enum Loop Complete.vi"("Current State Enum"=w360, "Itteration"=w358) -> ("Loop Complete?"=w359:bool)  [unwired: 12 in, 1 out]
    n175 = Increment(x=w360) -> (x+1=w367:T2)
  }
  n176 = for {
    tunnel: w2 -> [w387] mode=indexing
    tunnel: w1 -> [w386]
    n177 = call "Close ScrollZoomGraphChart.vi"("error in (no error)"=w386, "ScrollZoomGraphChart in"=w387) -> ()  [unwired: 9 in, 1 out]
  }
  n178 = disable-structure shown="RUN_TIME_ENGINE==True" {
    disable-tunnel: [w388 w389] -> w14
    disable-tunnel: w26 -> [w388 w390]
    frame condition #0 (active) {
    }
    frame condition #1 {
      n179 = flat-sequence {
        tunnel: [w391] -> w389
        tunnel: w390 -> [w391]
        frame #0 {
          n180 = Quit LabVIEW() -> ()  [unwired: 1 in]
        }
      }
    }
  }
  n181 = Unbundle By Name(w16) -> ("Terminate Error"=w15:errorcluster)
  n182 = Merge Errors(w15, w14) -> (→"error out":errorcluster)
  "top banner" <- u32 44412 ("top banner")
  "error background" <- u32 15461355 ("error background")
